vi "Overrid Dynamic Dispatch VIs.vi"(8 "error in (no error)":errorcluster, 11 "Mock Class Generator in":refnum<class "Mock Class Generator.lvclass">) -> (0 "error out":errorcluster, 2 "Created VI:s":path[](array[path]), 3 "Mock Class Generator out":refnum<class "Mock Class Generator.lvclass">)   [LabVIEW 2020, in "Mock Class Generator.lvclass"]
uses:
  Mock Class Generator.lvclass
  Mock Class Generator.lvclass/Mock Class Generator.ctl
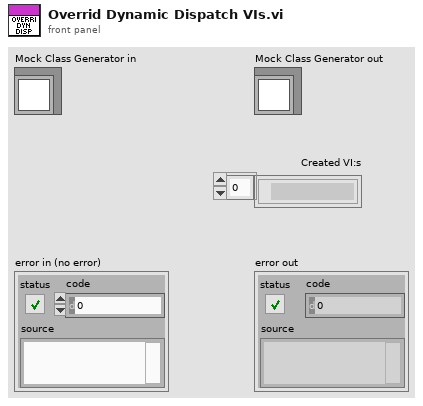
[diagram p1: front panel]
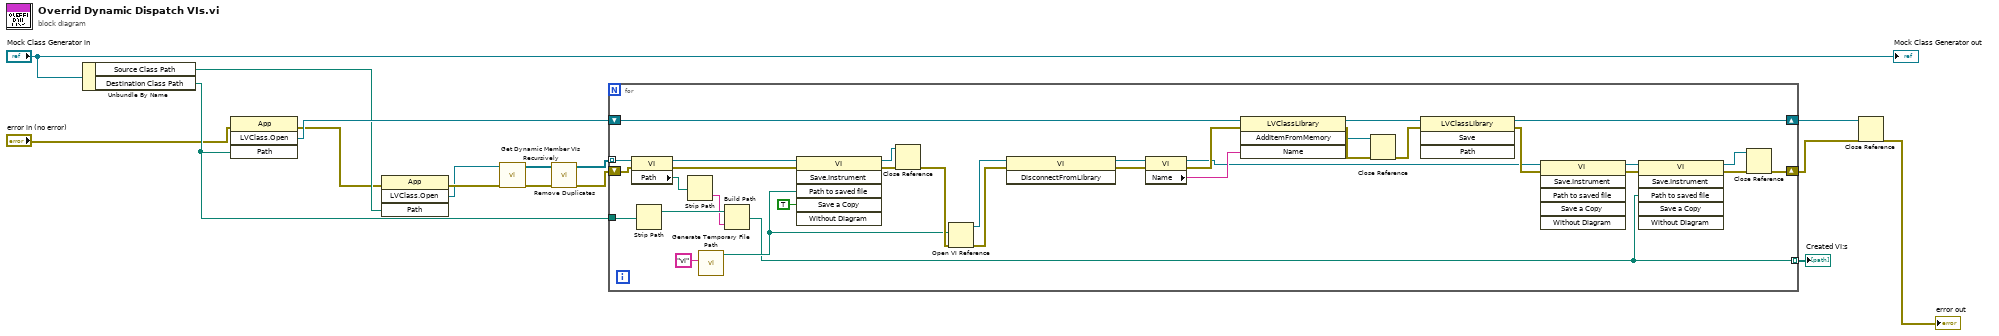
[diagram p0: block diagram]
diagram:
  n1 = Unbundle By Name("Mock Class Generator in") -> ("Source Class Path"=w6:path, "Destination Class Path"=w15:path)
  n2 = invoke class="App" method="LVClass.Open"(error in="error in (no error)", "Path"=w15) -> (error out=w4:errorcluster, "LVClass.Open"=w14:refnum<vi>)  [unwired: 2 in, 2 out]
  n3 = invoke class="App" method="LVClass.Open"(error in=w4, "Path"=w6) -> (error out=w5:errorcluster, "LVClass.Open"=w3:refnum<vi>)  [unwired: 2 in, 2 out]
  n4 = call "Get Dynamic Member VIs Recursively.vi"("error in (no error)"=w5, "Source Class"=w3) -> ("error out"=w10:errorcluster, "Dynamic Member VIs"=w9:refnum<vi>[])  [unwired: 8 in]
  n5 = call "Remove Duplicates.vi"("error in (no error)"=w10, "Dynamic Member VIs"=w9) -> ("error out"=w2:errorcluster, "Unique Dynamic Member VIs"=w1:refnum<vi>[])  [unwired: 8 in]
  n6 = for {
    tunnel: w1 -> [w50] mode=indexing
    shift-right: [w37] -> w11
    shift-left: w2 -> [w44]
    shift-right: [w35] -> w12
    shift-left: w14 -> [w42]
    tunnel: w15 -> [w23]
    tunnel: [w17] -> w7 mode=indexing
    n7 = property class="VI"(reference=w50, error in=w44) -> (reference out=w45:refnum<vi>, error out=w43:errorcluster, "Path"=w49:path)
    n8 = Strip Path(path=w23) -> (stripped path=w48:path)  [unwired: 1 out]
    n9 = Strip Path(path=w49) -> (name=w47:string)  [unwired: 1 out]
    n10 = call <vilib>:"Generate Temporary File Path.vi"("Temporary File Extension (tmp)"="vi") -> ("Unique Temporary File Path"=w21:path)  [unwired: 9 in, 1 out]
    n11 = Build Path(base path=w48, name or relative path=w47) -> (appended path=w17:path)
    n12 = invoke class="VI" method="Save.Instrument"(reference=w45, error in=w43, "Path to saved file"=w21, "Save a Copy"=TRUE) -> (reference out=w27:refnum<vi>, error out=w30:errorcluster)  [unwired: 2 in, 4 out]
    n13 = Close Reference(reference=w27, error in (no error)=w30) -> (error out=w26:errorcluster)
    n14 = Open VI Reference(vi path=w21, error in (no error)=w26) -> (vi reference=w25:refnum<vi>, error out=w24:errorcluster)  [unwired: 4 in]
    n15 = invoke class="VI" method="DisconnectFromLibrary"(reference=w25, error in=w24) -> (reference out=w28:refnum<vi>, error out=w29:errorcluster)  [unwired: 1 in, 1 out]
    n16 = property class="VI"(reference=w28, error in=w29) -> (reference out=w19:refnum<vi>, error out=w31:errorcluster, "Name"=w32:string)
    n17 = invoke class="LVClassLibrary" method="AddItemFromMemory"(reference=w42, error in=w31, "Name"=w32) -> (reference out=w36:refnum<vi>, error out=w41:errorcluster, "AddItemFromMemory"=w40:refnum<vi>)  [unwired: 1 in, 1 out]
    n18 = Close Reference(reference=w40, error in (no error)=w41) -> (error out=w34:errorcluster)
    n19 = invoke class="LVClassLibrary" method="Save"(reference=w36, error in=w34) -> (reference out=w35:refnum<vi>, error out=w33:errorcluster)  [unwired: 2 in, 2 out]
    n20 = invoke class="VI" method="Save.Instrument"(reference=w19, error in=w33) -> (reference out=w18:refnum<vi>, error out=w20:errorcluster)  [unwired: 4 in, 4 out]
    n21 = invoke class="VI" method="Save.Instrument"(reference=w18, error in=w20, "Path to saved file"=w17) -> (reference out=w39:refnum<vi>, error out=w38:errorcluster)  [unwired: 3 in, 4 out]
    n22 = Close Reference(reference=w39, error in (no error)=w38) -> (error out=w37:errorcluster)
  }
  "Created VI:s" <- w7
  n23 = Close Reference(reference=w12, error in (no error)=w11) -> (error out=→"error out":errorcluster)
  "Mock Class Generator out" <- "Mock Class Generator in"
